vi "create.vi"(8 "error in (no error)":errorcluster, 11 "path":path) -> (0 "error out":errorcluster, 3 "logging":refnum<class "system.logging.lvclass">)   [LabVIEW 2021, in "system.logging.lvclass"]
uses:
  system.logging.lvclass
  system.logging.lvclass/system.logging.ctl
panel:
  # "Create the logger and add it to the system container."
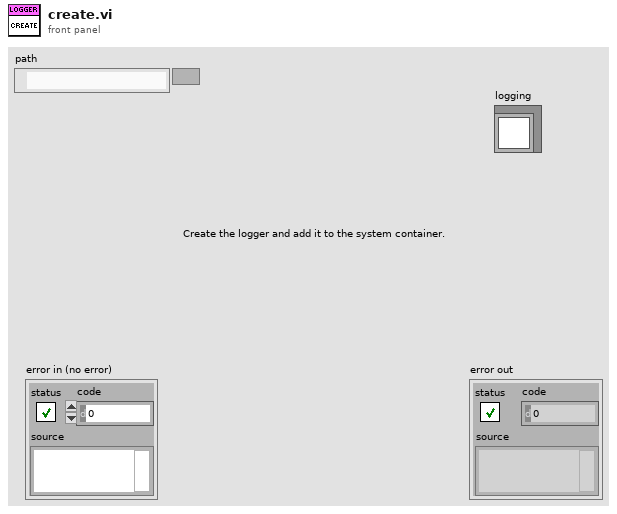
[diagram p1: front panel]
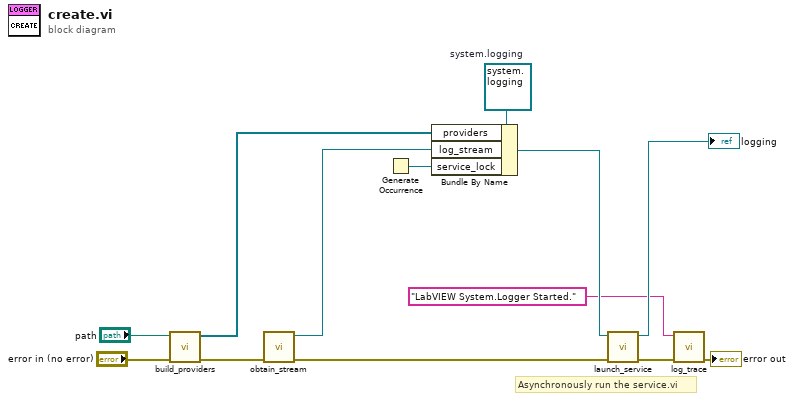
[diagram p0: block diagram]
diagram:
  w13 = refnum<class "system.logging.lvclass"> refnum  # system.logging
  # "Asynchronously run the service.vi"
  n1 = call "build_providers.vi"("error in"="error in (no error)", "path"="path") -> ("error out"=w11:errorcluster, "providers"=w10:refnum<class "system.logging.provider.lvclass">[])  [unwired: 8 in]
  n2 = call "obtain_stream.vi"("error in (no error)"=w11) -> ("error out"=w6:errorcluster, "log_stream"=w5:refnum<queue>)  [unwired: 9 in]
  n3 = Generate Occurrence() -> (w4:refnum<k4>)
  n4 = Bundle By Name(cluster=w13, "providers"=w10, "log_stream"=w5, "service_lock"=w4) -> (w8:refnum<class "system.logging.lvclass">)
  n5 = call "launch_service.vi"("error in (no error)"=w6, "system.logging in"=w8) -> ("error out"=w3:errorcluster, "system.logging out"=→"logging":refnum<class "system.logging.lvclass">)  [unwired: 8 in]
  n6 = call "log_trace.vi"("error in (no error)"=w3, "message"="LabVIEW System.Logger Started.") -> ("error out"=→"error out":errorcluster)  [unwired: 9 in]
